vi "TDMS Simple transference.vi"() -> ()   [LabVIEW 2016]
uses:
  <vilib>/WebDAVClient/Advanced/Get File.vi
  <vilib>/WebDAVClient/NI_WebDAV.lvlib
panel:
  out "Error out WebDAV Put @ cRIO":errorcluster
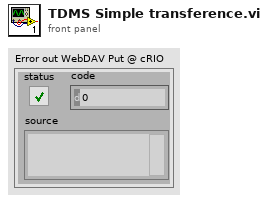
[diagram p1: front panel]
types:
  T1 = typedef "NI_WebDAV.lvlib/SessionHandle.ctl" = refnum<k1>
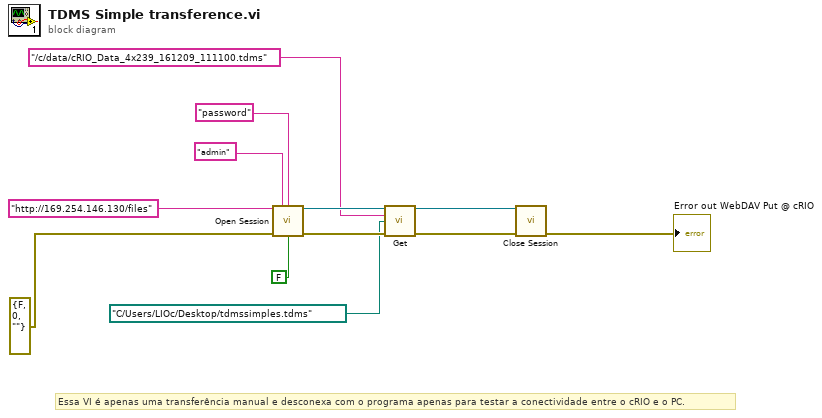
[diagram p0: block diagram]
diagram:
  # "Essa VI é apenas uma transferência manual e desconexa com o programa apenas para testar a conectividade entre o cRIO e o PC."
  n1 = call <vilib>:"Open Session.vi"("host uri prefix"="http://169.254.146.130/files", "username"="admin", "password"="password", "error in (no error)"=errorcluster {"status"=FALSE, "code"=0, "source"=""} ("error constant"), "verify server?"=FALSE) -> ("session handle out"=w10:T1, "error out"=w8:errorcluster)  [unwired: 9 in]
  n2 = call-poly <vilib>:"Get.vi"("session handle"=w10, "relative uri"="/c/data/cRIO_Data_4x239_161209_111100.tdms", "local file path"=path "C:/Users/LIOc/Desktop/tdmssimples.tdms", "error in (no error)"=w8) -> ("session handle out"=w9:T1, "error out"=w7:errorcluster)  [unwired: 9 in, 1 out]
  n3 = call <vilib>:"Close Session.vi"("session handle"=w9, "error in (no error)"=w7) -> ("error out"=→"Error out WebDAV Put @ cRIO":errorcluster)  [unwired: 13 in]
